vi "Display Module - Set Display Order.vi"(0 "Image Refs":T1[](array[typedef]), 11 "IMAQ Display Refs":refnum<vi>[](array[refnum])) -> ()   [LabVIEW 2021]
uses:
  <vilib>/vision/Image Controls.llb/IMAQ Image.ctl
  <vilib>/Utility/miscctls.llb/LVPointTypeDef.ctl
panel:
  in  "Cancel":bool
  in  "Reset":bool
  in  "Quit":bool
  # "Click on each image to change the order."
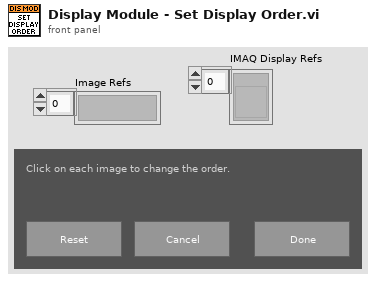
[diagram p1: front panel]
types:
  T1 = typedef "IMAQ Image.ctl" = refnum<image>
  T2 = enum8{"Enabled", "Disabled", "Disabled and Grayed Out"}
  T3 = enum16{"Always On", "Always Off", "Off While Running"}
  T4 = typedef "LVPointTypeDef.ctl" = cluster{"Horizontal":i16, "Vertical":i16}
  T5 = enum16{"User-specified Font", "Application Font", "System Font", "Dialog Font"}
  T6 = cluster{"Desired Font (Application)":enum16{"User-specified Font", "Application Font", "System Font", "Dialog Font"}, "[User-specified Font]":cluster{"Font Name":string, "Size":i16, "Strikeout?":bool, "Italic?":bool, "Underline?":bool, "Outline?":bool, "Shadow?":bool, "Bold?":bool, "Rotation Angle":dbl}, "Horizontal Alignment":i16, "Vertical Alignment":i16}
  T7 = cluster{"Font Name":string, "Size":i16, "Strikeout?":bool, "Italic?":bool, "Underline?":bool, "Outline?":bool, "Shadow?":bool, "Bold?":bool, "Rotation Angle":dbl}
  T8 = typedef "LVRectTypeDef.ctl" = cluster{"Left":i16, "Top":i16, "Right":i16, "Bottom":i16}
  T9 = typedef "LVBoundsTypeDef.ctl" = cluster{"Width":u32, "Height":u32}
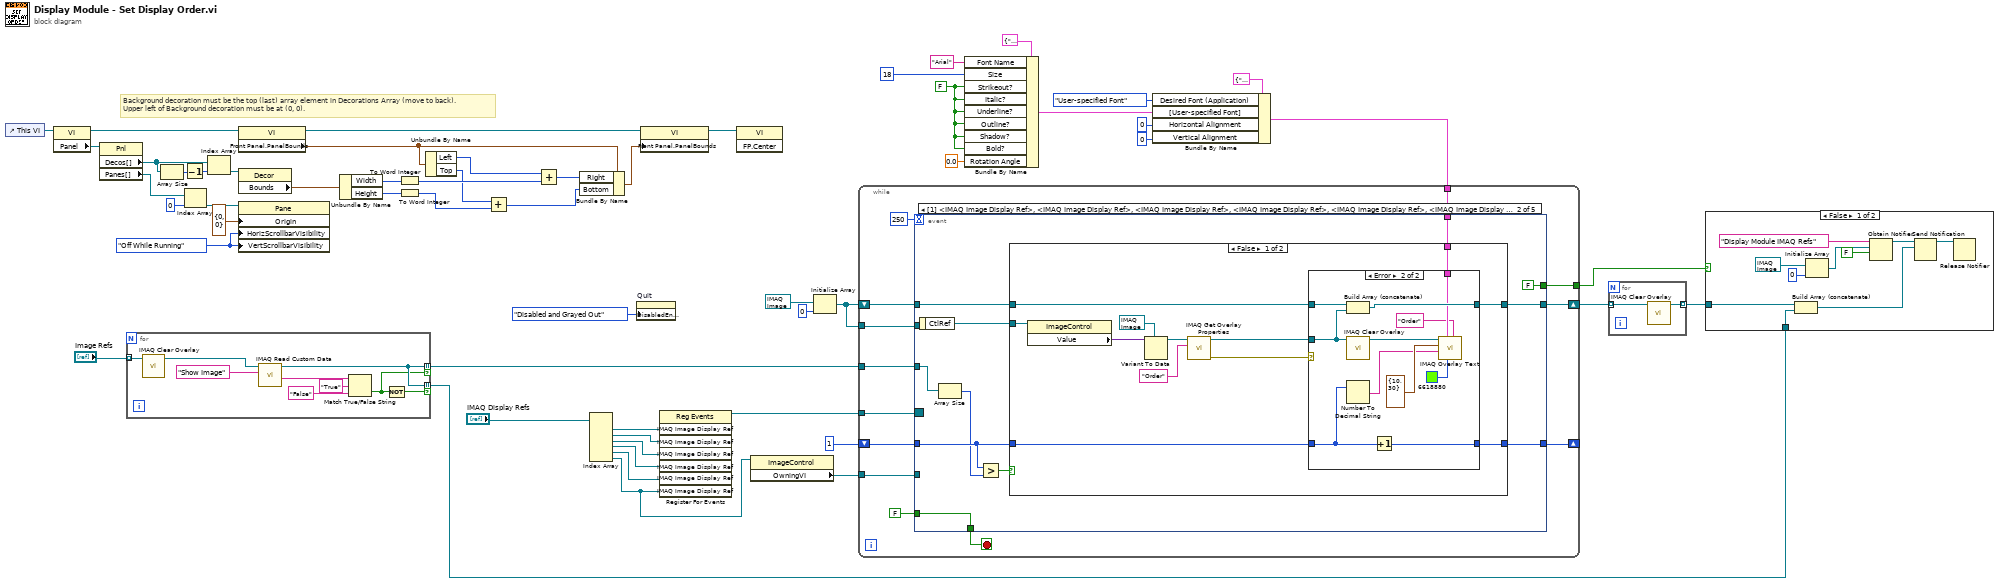
[diagram p0: block diagram]
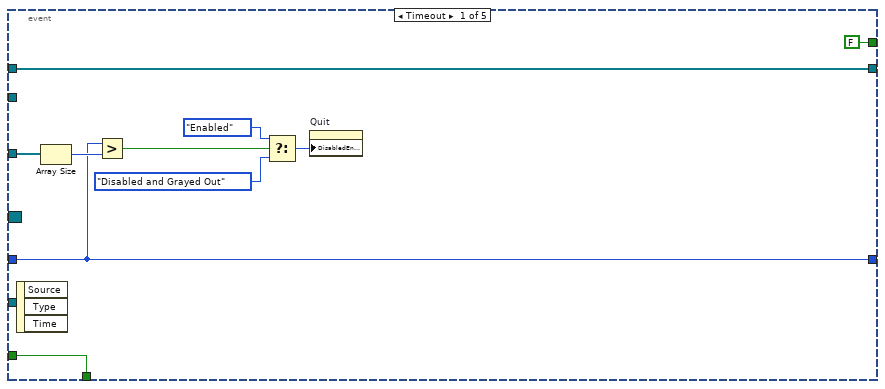
[diagram p3: hidden frame]
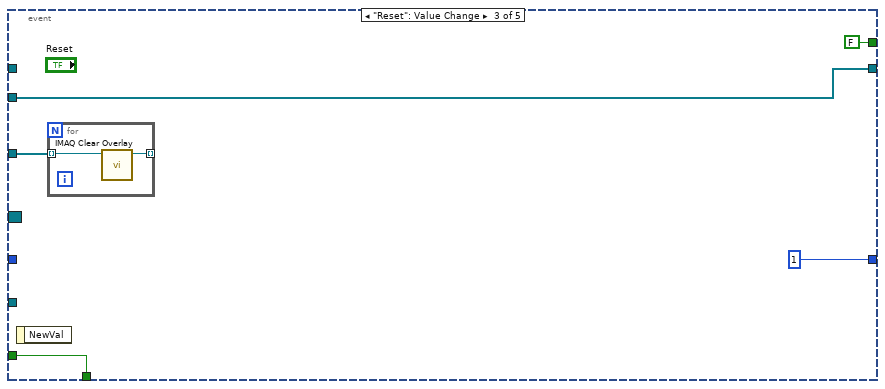
[diagram p6: hidden frame]
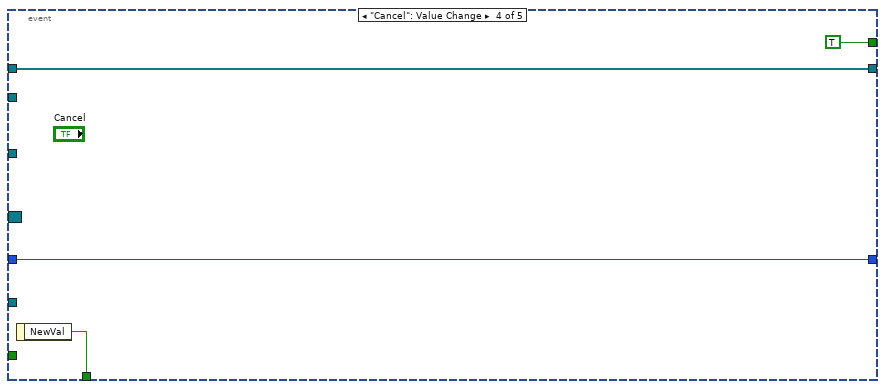
[diagram p7: hidden frame]
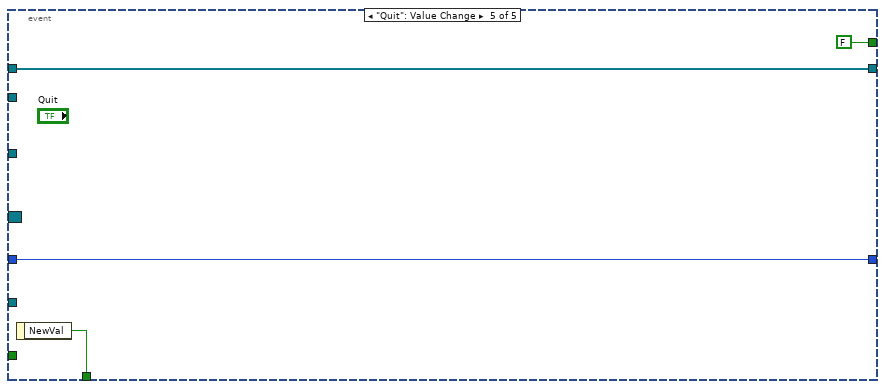
[diagram p8: hidden frame]
diagram:
  w20 = T3."Off While Running" ("Vertical Scrollbar Visibility")
  w32 = FALSE ("Strikeout?")
  # "Background decoration must be the top (last) array element in Decorations Array (move to back).\nUpper left of Background decoration must be at (0, 0)."
  n1 = control-ref of="This VI"() -> (w13:refnum<vi>)
  n2 = property class="VI"(reference=w13) -> (reference out=w21:refnum<vi>, "Panel"=w14:refnum<vi>)  [unwired: 1 in, 1 out]
  n3 = property class="Pnl"(reference=w14) -> ("Decos[]"=w12:refnum<vi>[], "Panes[]"=w17:refnum<vi>[])  [unwired: 1 in, 2 out]
  n4 = for {
    tunnel: "Image Refs" -> [w61] mode=indexing
    tunnel: [w59] -> w43 mode=indexing if=w58
    tunnel: [w59] -> w42 mode=indexing if=w57
    n5 = call "IMAQ Clear Overlay"("Image"=w61) -> ("Image Out"=w60:T1)  [unwired: 9 in, 1 out]
    n6 = call "IMAQ Read Custom Data"("Key"="Show Image", "Image"=w60) -> ("Custom Data Out"=w65:string, "Image (duplicate)"=w59:T1)  [unwired: 7 in, 1 out]
    n7 = Match True/False String(2:"False" ("false string"), 3:"True" ("true string"), 4:w65) -> (0:w58:bool)  [unwired: 1 out]
    n8 = Not(x=w58) -> (.not. x?=w57:bool)
  }
  n9 = Array Size(array=w12) -> (size(s)=w10:i32)
  n10 = Decrement(x=w10) -> (x-1=w11:i32)
  n11 = Index Array(array=w17, index=0) -> (element=w16:refnum<vi>)
  n12 = Index Array(array=w12, index=w11) -> (element=w19:refnum<vi>)
  n13 = property class="VI"(reference=w21) -> (reference out=w23:refnum<vi>, "Front Panel.PanelBounds"=w24:T8)  [unwired: 1 in, 1 out]
  n14 = property class="Decor"(reference=w19) -> ("Bounds"=w22:T9)  [unwired: 1 in, 2 out]
  n15 = property class="Pane"(reference=w16, "Origin"=T4 {"Horizontal"=0, "Vertical"=0}, "HorizScrollbarVisibility"=w20, "VertScrollbarVisibility"=w20) -> ()  [unwired: 1 in, 2 out]
  n16 = Unbundle By Name(w22) -> ("Width"=w27:u32, "Height"=w30:u32)
  n17 = To Word Integer(number=w27) -> (16bit integer=w29:i16)
  n18 = To Word Integer(number=w30) -> (16bit integer=w8:i16)
  n19 = Unbundle By Name(w24) -> ("Left"=w26:i16, "Top"=w9:i16)
  n20 = Add(x=w9, y=w8) -> (x+y=w7:i16)
  n21 = Add(x=w26, y=w29) -> (x+y=w28:i16)
  n22 = Bundle By Name(cluster=w24, "Right"=w28, "Bottom"=w7) -> (w25:T8)
  n23 = Index Array(array="IMAQ Display Refs") -> (element #1=w51:refnum<vi>, element #2=w55:refnum<vi>, element #3=w52:refnum<vi>, element #4=w53:refnum<vi>, element #5=w54:refnum<vi>, element #6=w48:refnum<vi>)  [unwired: 6 in]
  n24 = property on="Quit" class="Bool"("DisabledEnum"=T2."Disabled and Grayed Out" ("Disabled")) -> ()  [unwired: 2 in, 2 out]
  n25 = property class="VI"(reference=w23, "Front Panel.PanelBounds"=w25) -> (reference out=w6:refnum<vi>)  [unwired: 1 in, 1 out]
  n26 = register-events(w51, w55, w52, w53, w54, w48) -> (reference out=w50:refnum<event-registration>)  [unwired: 2 in, 1 out]
  n27 = invoke class="VI" method="FP.Center"(reference=w6) -> ()  [unwired: 2 in, 3 out]
  n28 = property class="ImageControl"(reference=w48) -> ("OwningVI"=w47:refnum<vi>)  [unwired: 1 in, 2 out]
  n29 = Initialize Array(T1 refnum ("New Image"), 0 ("dimension size")) -> (w3:T1[])
  n30 = Bundle By Name(cluster=T7 {"Font Name"="", "Size"=0, "Strikeout?"=FALSE, "Italic?"=FALSE, "Underline?"=FALSE, "Outline?"=FALSE, "Shadow?"=FALSE, "Bold?"=FALSE, "Rotation Angle"=0.0} ("[User-specified Font]"), "Font Name"="Arial", "Size"=i16 18, "Strikeout?"=w32, "Italic?"=w32, "Underline?"=w32, "Outline?"=w32, "Shadow?"=w32, "Bold?"=w32, "Rotation Angle"=0.0) -> (w34:T7)
  n31 = Bundle By Name(cluster=T6 {"Desired Font (Application)"=enum."Application Font", "[User-specified Font]"={"Font Name"="", "Size"=12, "Strikeout?"=FALSE, "Italic?"=FALSE, "Underline?"=FALSE, "Outline?"=FALSE, "Shadow?"=FALSE, "Bold?"=FALSE, "Rotation Angle"=0.0}, "Horizontal Alignment"=0, "Vertical Alignment"=0} ("Font, Size & Style"), "Desired Font (Application)"=T5."User-specified Font", "[User-specified Font]"=w34, "Horizontal Alignment"=i16 0, "Vertical Alignment"=i16 0) -> (w31:T6)
  n32 = while {
    tunnel: w50 -> [w75]
    shift-right: [w73] -> _
    shift-left: 1 -> [w74]
    tunnel: w47 -> [w72]
    tunnel: w43 -> [w70]
    shift-right: [w69] -> w5
    shift-left: w3 -> [w71]
    tunnel: w31 -> [w68]
    tunnel: w3 -> [w67]
    tunnel: [w66] -> w1
    stop <- w78 stop-if-true
    n33 = event shown="[1] <IMAQ Image Display Ref>, <IMAQ Image Display Ref>, <IMAQ Image Display Ref>, <IMAQ Image Display Ref>, <IMAQ Image Display Ref>, <IMAQ Image Display Ref>: Mouse Down" {
      selector: w75 -> [_ _ _ _ _]
      dyn-events: _ -> [_ _ _ _ _]
      timeout: 250 -> [_ _ _ _ _]
      tunnel: [w88 w99 w131 w137 w141] -> w78
      tunnel: FALSE -> [w88 w99 w131 _ _]
      tunnel: w74 -> [w84 w97 _ w136 w140]
      tunnel: [w84 w95 1 w136 w140] -> w73
      tunnel: w72 -> [_ _ _ _ _]
      tunnel: w71 -> [w87 w94 _ w135 w139]
      tunnel: w70 -> [w85 w93 w129 _ _]
      tunnel: [w87 w91 w128 w135 w139] -> w69
      tunnel: w68 -> [_ w90 _ _ _]
      tunnel: w67 -> [_ _ w128 _ _]
      tunnel: [FALSE FALSE FALSE TRUE FALSE] -> w66
      event Timeout {
        n34 = event-data() -> ()  [unwired: 1 in, 3 out]
        n35 = Array Size(array=w85) -> (size(s)=w86:i32)
        n36 = Greater?(x=w84, y=w86) -> (0:w83:bool)
        n37 = Select(t=T2."Enabled" ("Disabled"), s=w83, f=T2."Disabled and Grayed Out" ("Disabled")) -> (s? t:f=w81:T2)
        n38 = property on="Quit" class="Bool"("DisabledEnum"=w81) -> ()  [unwired: 2 in, 2 out]
      }
      event Mouse Down {
        n39 = event-data() -> ("CtlRef"=w96:refnum<vi>)  [unwired: 1 in]
        n40 = Array Size(array=w93) -> (size(s)=w92:i32)
        n41 = Greater?(x=w97, y=w92) -> (0:w98:bool)
        n42 = case shown="False" w98 {
          tunnel: w97 -> [w104 w126]
          tunnel: w96 -> [w110 _]
          tunnel: [w111 w126] -> w95
          tunnel: w94 -> [w109 w125]
          tunnel: [w106 w125] -> w91
          tunnel: w90 -> [w105 _]
          frame False {
            n43 = property class="ImageControl"(reference=w110) -> ("Value"=w108:variant)  [unwired: 1 in, 2 out]
            n44 = Variant To Data(type=T1 refnum ("New Image"), Variant=w108) -> (data=w103:T1)  [unwired: 1 in, 1 out]
            n45 = call "IMAQ Get Overlay Properties"("Group"="Order", "Image"=w103) -> ("error out"=w101:errorcluster, "Image Out"=w102:T1)  [unwired: 5 in, 1 out]
            n46 = case shown="Error" w101 {
              tunnel: [w112 w124] -> w111
              tunnel: w109 -> [w113 w123]
              tunnel: [w113 w122] -> w106
              tunnel: w105 -> [_ w119]
              tunnel: w104 -> [w112 w118]
              tunnel: w102 -> [_ w116]
              frame No Error {
              }
              frame Error {
                n47 = Build Array (concatenate)(w123, w116) -> (w122:T1[])
                n48 = call "IMAQ Clear Overlay"("Image"=w116) -> ("Image Out"=w115:T1)  [unwired: 9 in, 1 out]
                n49 = Number To Decimal String(number=w118) -> (decimal integer string=w117:string)  [unwired: 1 in]
                n50 = Increment(x=w118) -> (x+1=w124:i32)
                n51 = call "IMAQ Overlay Text"("Group"="Order", "Text Color (black)"=u32 6618880, "Font, Size & Style"=w119, "String"=w117, "Origin"=cluster{"X":i32, "Y":i32} {"X"=10, "Y"=30}, "Image"=w115) -> ()  [unwired: 4 in, 2 out]
              }
            }
          }
          frame True {
          }
        }
      }
      event "Reset": Value Change {
        n52 = event-data() -> ()  [unwired: 1 in, 1 out]
        n53 = for {
          tunnel: w129 -> [w133] mode=indexing
          tunnel: [w132] -> _ mode=indexing
          n54 = call "IMAQ Clear Overlay"("Image"=w133) -> ("Image Out"=w132:T1)  [unwired: 9 in, 1 out]
        }
      }
      event "Cancel": Value Change {
        n55 = event-data() -> ("NewVal"=w137:bool)  [unwired: 1 in]
      }
      event "Quit": Value Change {
        n56 = event-data() -> ("NewVal"=w141:bool)  [unwired: 1 in]
      }
    }
  }
  n57 = for {
    tunnel: w5 -> [w143] mode=indexing
    tunnel: [w142] -> w2 mode=indexing
    n58 = call "IMAQ Clear Overlay"("Image"=w143) -> ("Image Out"=w142:T1)  [unwired: 9 in, 1 out]
  }
  n59 = case shown="False" w1 {
    tunnel: w42 -> [w153 _]
    tunnel: w2 -> [w152 _]
    frame False {
      n60 = Build Array (concatenate)(w152, w153) -> (w145:T1[])
      n61 = Initialize Array(T1 refnum ("New Image"), 0 ("dimension size")) -> (w147:T1[])
      n62 = Obtain Notifier(name (unnamed)="Display Module IMAQ Refs", notification data type=w147, create if not found? (T)=FALSE) -> (notifier out=w146:refnum<notifier>)  [unwired: 1 in, 2 out]
      n63 = Send Notification(notification=w145, notifier=w146) -> (notifier out=w144:refnum<notifier>)  [unwired: 1 in, 1 out]
      n64 = Release Notifier(notifier=w144) -> ()  [unwired: 2 in, 3 out]
    }
    frame True {
    }
  }
